vi "Open.vi"(6 "VI":refnum<vi>, 7 "Delay mSec (0)":u32, 8 "error in (no error)":errorcluster, 9 "Explorer Visible? (F)":bool, 10 "Process Events Registration":refnum<event-registration>, 11 "Window Title":string="Action Status") -> (0 "error out":errorcluster, 2 "UI Events Registration":refnum<event-registration>)   [LabVIEW 2015]
uses:
  Simple Progress Bar.lvlib
  Process Events.ctl
  UI Events.ctl
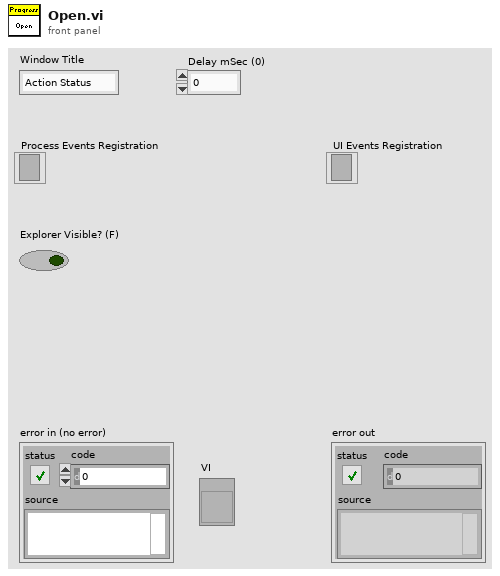
[diagram p1: front panel]
types:
  T1 = enum32{"Invalid", "Standard", "Closed", "Hidden", "Minimized", "Maximized"}
  T2 = typedef "Simple Progress Bar.lvlib/UI Events.ctl" = cluster{"Done":refnum<user-event>, "Cancel":refnum<user-event>, "Explore":refnum<user-event>}
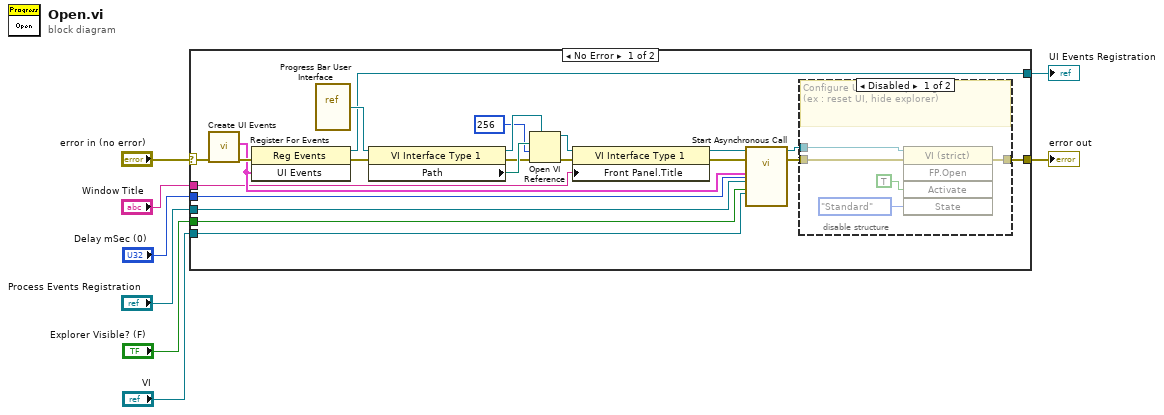
[diagram p0: block diagram]
diagram:
  n1 = case shown="No Error" "error in (no error)" {
    selector: "error in (no error)" -> [w19 w37]
    tunnel: [w24 w37] -> w7
    tunnel: [w18 _] -> w6
    tunnel: "Explorer Visible? (F)" -> [w17 _]
    tunnel: "Process Events Registration" -> [w16 _]
    tunnel: "Window Title" -> [w11 _]
    tunnel: "VI" -> [w10 _]
    tunnel: "Delay mSec (0)" -> [w9 _]
    frame No Error {
      n2 = call "Create UI Events.vi"("error in (no error)"=w19) -> ("error out"=w22:errorcluster, "UI Events"=w20:T2)  [unwired: 9 in]
      n3 = register-events(error in=w22, w20) -> (reference out=w18:refnum<event-registration>, error out=w21:errorcluster)  [unwired: 1 in]
      n4 = vi-ref "Progress Bar User Interface.vi"() -> (w30:refnum<vi>)
      n5 = property class="VI Interface Type 1"(reference=w30, error in=w21) -> (reference out=w27:refnum<vi>, error out=w28:errorcluster, "Path"=w29:path)
      n6 = Open VI Reference(type specifier VI Refnum (for type only)=w27, vi path=w29, options=256, error in (no error)=w28) -> (vi reference=w13:refnum<vi>, error out=w26:errorcluster)  [unwired: 2 in]
      n7 = property class="VI Interface Type 1"(reference=w13, error in=w26, "Front Panel.Title"=w11) -> (reference out=w12:refnum<vi>, error out=w14:errorcluster)
      n8 = call-by-ref "Start Asynchronous Call"(reference=w12, error in=w14, "VI"=w10, "Delay mSec (0)"=w9, "Explorer Visible? (F)"=w17, "Process Events Registration"=w16, "UI Events"=w20) -> (reference out=w23:refnum<vi>, error out=w25:errorcluster)  [unwired: 5 in, 2 out]
      n9 = disable-structure shown="Disabled" {
        disable-tunnel: w25 -> [w35 w36]
        disable-tunnel: [w34 w36] -> w24
        disable-tunnel: w23 -> [w33 _]
        frame Disabled {
          # "Configure UI before opening.\n(ex : reset UI, hide explorer)"
          n10 = invoke class="VI (strict)" method="FP.Open"(reference=w33, error in=w35, "Activate"=TRUE ("Activate?"), "State"=T1."Standard") -> (error out=w34:errorcluster)  [unwired: 1 in, 4 out]
        }
        frame Enabled {
        }
      }
    }
    frame Error {
    }
  }
  "error out" <- w7
  "UI Events Registration" <- w6
